vi "Startup Dialog.vi"(8 "error in":errorcluster) -> (0 "error out":errorcluster)   [LabVIEW 2025, in "I2C Bus Monitor UI.lvlib"]
uses:
  I2C Bus Monitor UI.lvlib
  <vilib>/Utility/config.llb/Read Key (Boolean).vi
  Error Global.vi
  <vilib>/Utility/config.llb/Write Key (Boolean).vi
  <vilib>/Utility/config.llb/NI_LVConfig.lvlib
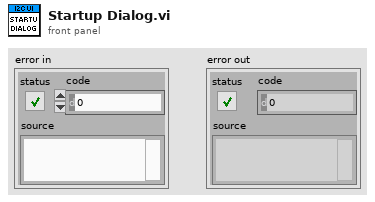
[diagram p1: front panel]
types:
  T1 = typedef "NI_LVConfig.lvlib/Config Data RefNum.ctl" = refnum<k1>
  T2 = enum16{"Left Button", "Center Button", "Right Button", "Window Close"}
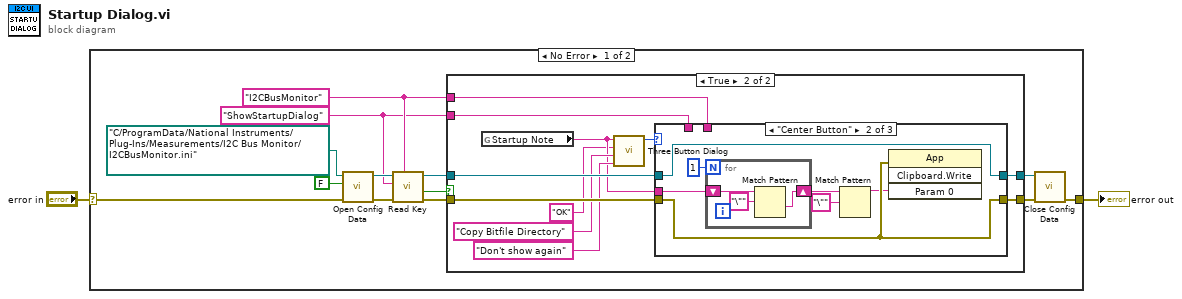
[diagram p0: block diagram]
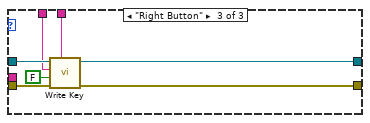
[diagram p4: hidden frame]
diagram:
  n1 = case shown="No Error" "error in" {
    selector: "error in" -> [w14 w48]
    tunnel: [w7 w48] -> w1
    frame No Error {
      w5 = "I2CBusMonitor" ("section")
      w4 = "ShowStartupDialog" ("key")
      n2 = call <vilib>:"Open Config Data.vi"("error in (no error)"=w14, "create file if necessary (T)"=FALSE, "configuration file path"=path "C:/ProgramData/National Instruments/Plug-Ins/Measurements/I2C Bus Monitor/I2CBusMonitor.ini") -> ("error out"=w13:errorcluster, "refnum"=w12:T1)  [unwired: 6 in, 1 out]
      n3 = call-poly <vilib>:"Read Key.vi"("section"=w5, "error in (no error)"=w13, "key"=w4, "refnum"=w12) -> ("error out"=w10:errorcluster, "value"=w9:bool, "refnum out"=w8:T1)  [unwired: 4 in, 1 out]
      n4 = case shown="True" w9 {
        tunnel: [w17 w28] -> w15
        tunnel: w10 -> [w17 w27]
        tunnel: w8 -> [w16 w25]
        tunnel: [w16 w24] -> w6
        tunnel: w5 -> [_ w23]
        tunnel: w4 -> [_ w22]
        frame False {
        }
        frame True {
          n5 = global read "Error Global.vi" "Startup Note"() -> (w19:string)
          n6 = call <vilib>:"Three Button Dialog.vi"("Right Button Text (\"Cancel\")"="Don't show again" ("F button name (\"Cancel\")"), "Center Button Text (\"No\")"="Copy Bitfile Directory" ("F button name (\"Cancel\")"), "Left Button Text (\"Yes\")"="OK" ("Left Button Text (\"Yes\")"), "message"=w19) -> ("Which Button?"=w26:T2)  [unwired: 7 in]
          n7 = case shown="\"Center Button\"" w26 {
            tunnel: [w30 w37 w46] -> w28
            tunnel: w27 -> [w30 w37 w47]
            tunnel: w25 -> [w29 w36 w45]
            tunnel: [w29 w36 w44] -> w24
            tunnel: w23 -> [_ _ w43]
            tunnel: w22 -> [_ _ w42]
            tunnel: w19 -> [_ w31 _]
            frame "Left Button", Default {
            }
            frame "Center Button" {
              n8 = for {
                N: 1 -> [_]
                shift-right: [w38] -> w34
                shift-left: w31 -> [w40]
                n9 = Match Pattern(string=w40, regular expression="\"") -> (after substring=w38:string)  [unwired: 1 in, 3 out]
              }
              n10 = Match Pattern(string=w34, regular expression="\"") -> (before substring=w35:string)  [unwired: 1 in, 3 out]
              n11 = invoke class="App" method="Clipboard.Write"(error in=w37, "Param 0"=w35) -> ()  [unwired: 2 in, 4 out]
            }
            frame "Right Button" {
              n12 = call-poly <vilib>:"Write Key.vi"("section"=w43, "error in (no error)"=w47, "value"=FALSE, "key"=w42, "refnum"=w45) -> ("error out"=w46:errorcluster, "refnum out"=w44:T1)  [unwired: 4 in, 1 out]
            }
          }
        }
      }
      n13 = call <vilib>:"Close Config Data.vi"("error in (no error)"=w15, "refnum"=w6) -> ("error out"=w7:errorcluster)  [unwired: 8 in, 1 out]
    }
    frame Error {
    }
  }
  "error out" <- w1
